vi "VIH HelpGen - Build HTML Help.vi"(6 "Allowed files (empty=all)":path[](array[path]), 8 "error in":errorcluster, 9 "File paths":path[](array[path]), 10 "Menu paths":path[](array[path]), 11 "Project Tree":T1) -> (0 "error out":errorcluster, 3 "dup Project Tree":T1)   [LabVIEW 2014]
doc: "::: VI Helpeks :::\nCopyright (c) 2000-2026 Konstantin Shifershteyn. All rights reserved."
uses:
  _VIH Project Manager.llb/VIH Project Tree Typedef - Tree Refnum.ctl
  _VIH HelpGen - Palette.llb/VIH HelpGen Typedef - Palette - Item Info Cluster.ctl
  _VIH HelpGen - Palette.llb/VIH HelpGen Typedef - Palette - Item Type Enum.ctl
panel:
  # "VI Helpeks\nCopyright (c) 2012-2026 Konstantin Shifershteyn"
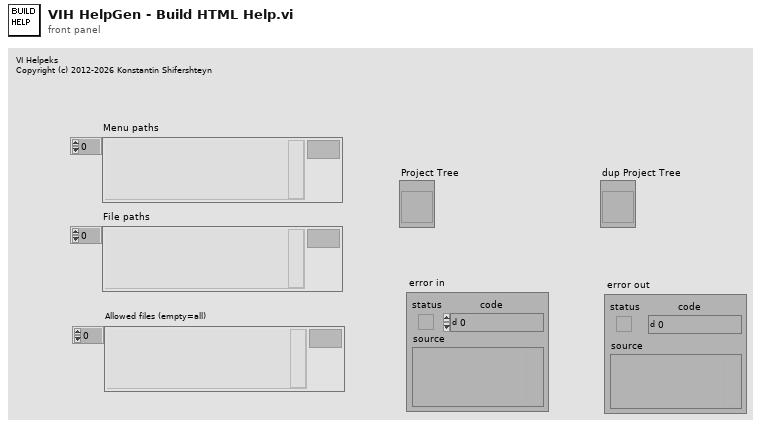
[diagram p1: front panel]
types:
  T1 = typedef "VIH Project Tree Typedef - Tree Refnum.ctl" = refnum<vi>
  T2 = enum16{"nop", "Start", "Stop", "Run-prep", "Run-VI", "Run-Menu"}
  T3 = typedef "VIH HelpGen Typedef - Palette - Item Info Cluster.ctl" = cluster{"Item Type":T4, "Item Name":string, "Item File":path, "Parent palette":path, "Not found":bool}
  T4 = typedef "VIH HelpGen Typedef - Palette - Item Type Enum.ctl" = enum32{"<Invalid>", "<unknown>", "VI", "Menu", "LV Func", "Express VI", "Poly VI", "CTL", "HTML"}
  T5 = cluster{"Show Window":bool, "Show Progress":bool, "Generate HTML":bool, "Generate HHP":bool, "Generate CHM":bool}
  T6 = typedef "VIH - CHM Project - HHP Generation Params Cluster.ctl" = cluster{"HHP_Template":enum16{"default", "custom"}, "HHP_Template_CustomPath":path, "HHP_Target":enum16{"default", "custom"}, "HHP_Target_CustomPath":path, "HHP_CreateTOC":bool, "HHP_CreateIDX":bool, "HHP_DefaultTopic":enum16{"auto", "custom"}, "HHP_DefaultTopic_CustomPath":path, "CHM_Filename":path, "HHP_AutoBuild":bool, "CHM_AutoBuild":bool}
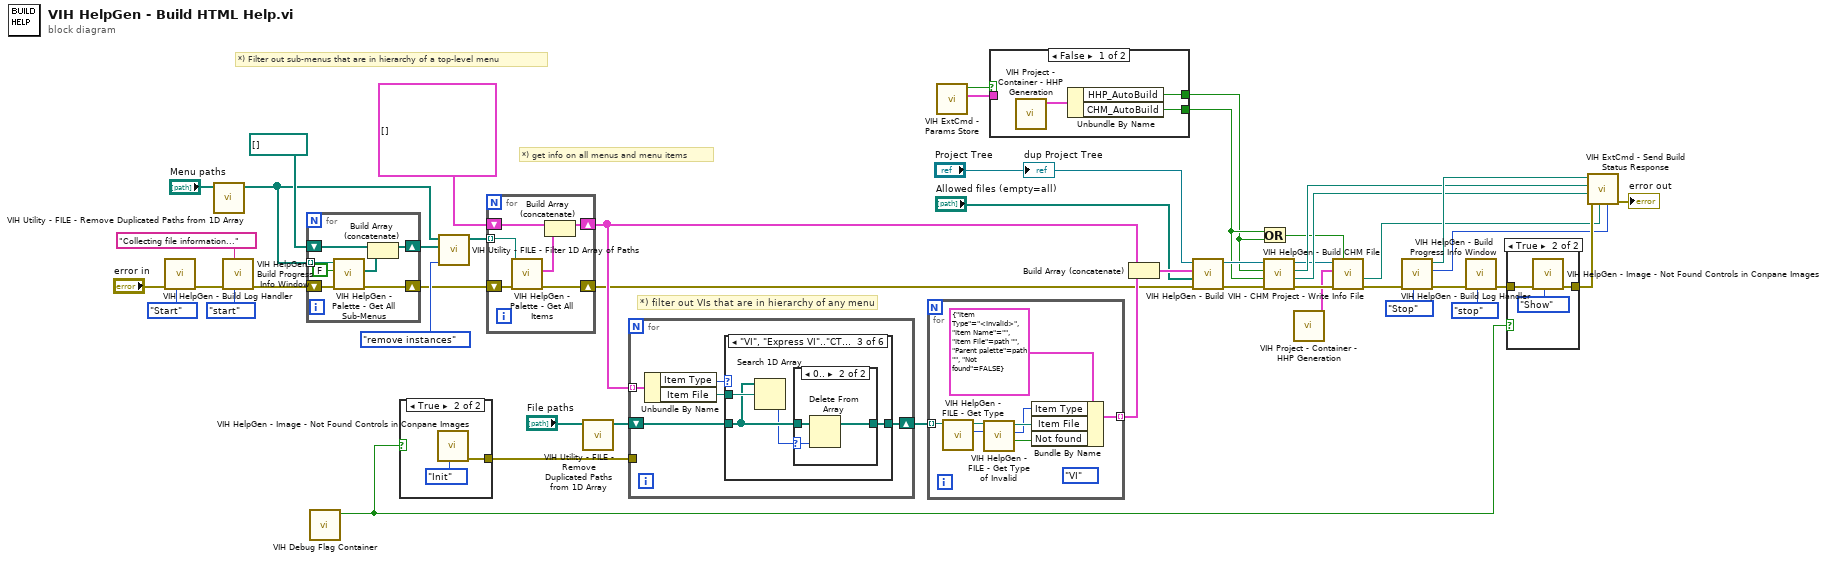
[diagram p0: block diagram]
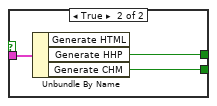
[diagram p2: hidden frame]
diagram:
  # "*) filter out VIs that are in hierarchy of any menu"
  # "*) get info on all menus and menu items"
  # "*) Filter out sub-menus that are in hierarchy of a top-level menu"
  n1 = call "VIH HelpGen - Build Log Handler.vi"("cmd (nop)"=T2."Start" ("cmd"), "error in"="error in") -> ("error out"=w35:errorcluster)  [unwired: 5 in, 4 out]
  n2 = call "VIH Utility - FILE - Remove Duplicated Paths from 1D Array.vi"("Array in"="Menu paths") -> ("Array out"=w28:path[])  [unwired: 9 in, 1 out]
  n3 = call "VIH HelpGen - Build Progress Info Window.vi"("Mode (run1)"=enum16{"start", "stop", "run1", "run2"}."start" ("Mode (run)"), "Message"="Collecting file information...", "error in"=w35) -> ("error out"=w33:errorcluster)  [unwired: 8 in]
  n4 = for {
    tunnel: w28 -> [w54] mode=indexing
    shift-right: [w51] -> w32
    shift-left: path[] [] -> [w52]
    shift-right: [w49] -> w27
    shift-left: w33 -> [w50]
    n5 = call "VIH HelpGen - Palette - Get All Sub-Menus.vi"("error in"=w50, "Include master menu (T)"=FALSE, "Palette Path"=w54) -> ("error out"=w49:errorcluster, "Palette Paths"=w53:path[])  [unwired: 7 in]
    n6 = Build Array (concatenate)(w52, w53) -> (w51:path[])
  }
  n7 = call "VIH Debug Flag Container.vi"() -> ("Debug Mode"=w23:bool)  [unwired: 11 in]
  n8 = case shown="True" w23 {
    tunnel: [_ w55] -> w26
    frame False {
    }
    frame True {
      n9 = call "VIH HelpGen - Image - Not Found Controls in Conpane Images.vi"("cmd"=enum16{"nop", "Init", "Add", "Show"}."Init") -> ("error out"=w55:errorcluster)  [unwired: 10 in]
    }
  }
  n10 = call "VIH Utility - FILE - Filter 1D Array of Paths.vi"("Action (keep instances)"=enum16{"keep instances", "remove instances"}."remove instances", "Instances"=w32, "Paths in"=w28) -> ("Paths out"=w29:path[])  [unwired: 4 in]
  n11 = for {
    shift-right: [w60] -> w39
    shift-left: w27 -> [w62]
    tunnel: w29 -> [w61] mode=indexing
    shift-right: [w57] -> w45
    shift-left: T3[] [] -> [w58]
    n12 = call "VIH HelpGen - Palette - Get All Items.vi"("error in"=w62, "Palette Path"=w61) -> ("error out"=w60:errorcluster, "Items Array"=w59:T3[])  [unwired: 7 in, 1 out]
    n13 = Build Array (concatenate)(w58, w59) -> (w57:T3[])
  }
  n14 = call "VIH Utility - FILE - Remove Duplicated Paths from 1D Array.vi"("Array in"="File paths") -> ("Array out"=w40:path[])  [unwired: 9 in, 1 out]
  n15 = for {
    tunnel: w45 -> [w67] mode=indexing
    shift-right: [w63] -> w46
    shift-left: w40 -> [w64]
    tunnel: w26 -> [_]
    n16 = Unbundle By Name(w67) -> ("Item Type"=w66:T4, "Item File"=w65:path)
    n17 = case shown="\"VI\", \"Express VI\"..\"CTL\"" w66 {
      tunnel: w65 -> [_ _ w73 _ _ _]
      tunnel: w64 -> [w68 w69 w72 w78 w79 w80]
      tunnel: [w68 w69 w71 w78 w79 w80] -> w63
      frame "<Invalid>" {
      }
      frame "<unknown>" {
      }
      frame "VI", "Express VI".."CTL" {
        n18 = Search 1D Array(1D array=w72, element=w73) -> (index of element=w70:i32)  [unwired: 1 in]
        n19 = case shown="0.." w70 {
          selector: w70 -> [_ w75]
          tunnel: w72 -> [w74 w77]
          tunnel: [w74 w76] -> w71
          frame ..-1 {
          }
          frame 0.. {
            n20 = Delete From Array "Delete From Array"(array=w77, index=w75) -> (array with subset deleted=w76:path[])  [unwired: 1 in, 1 out]
          }
        }
      }
      frame "Menu" {
      }
      frame "LV Func" {
      }
      frame "HTML" {
      }
    }
  }
  n21 = for {
    tunnel: w46 -> [w87] mode=indexing
    tunnel: [w88] -> w44 mode=indexing
    (unwired) VIH_HelpGen_Typedef_-_Palette_-_Item_Type_Enum."VI" ("Item Type")
    n22 = call "VIH HelpGen - FILE - Get Type.vi"("File Path"=w87) -> ("File Type"=w84:T4, "dup File Path"=w85:path)  [unwired: 8 in, 1 out]
    n23 = call "VIH HelpGen - FILE - Get Type of Invalid.vi"("File Type"=w84, "File Path"=w85) -> ("Not found"=w82:bool, "File Type out"=w81:T4, "File Path out"=w83:path)  [unwired: 6 in, 1 out]
    n24 = Bundle By Name(cluster=T3 {"Item Type"=enum."<Invalid>", "Item Name"="", "Item File"=path "", "Parent palette"=path "", "Not found"=FALSE} ("Item Info"), "Item Type"=w81, "Item File"=w83, "Not found"=w82) -> (w88:T3)
  }
  n25 = call "VIH ExtCmd - Params Store.vi"() -> ("Params"=w15:T5, "Ext Command"=w12:bool)  [unwired: 10 in]
  n26 = case shown="False" w12 {
    tunnel: w15 -> [_ w94]
    tunnel: [w90 w93] -> w3
    tunnel: [w89 w92] -> w4
    frame False {
      n27 = call "VIH Project - Container - HHP Generation.vi"() -> ("HHP_Generation out"=w91:T6)  [unwired: 11 in]
      n28 = Unbundle By Name(w91) -> ("HHP_AutoBuild"=w90:bool, "CHM_AutoBuild"=w89:bool)
    }
    frame True {
      n29 = Unbundle By Name(w94) -> ("Generate HHP"=w93:bool, "Generate CHM"=w92:bool)  [unwired: 1 out]
    }
  }
  n30 = Build Array (concatenate)(w45, w44) -> (w25:T3[])
  n31 = call "VIH HelpGen - Build.vi"("error in"=w39, "Allowed files"="Allowed files (empty=all)", "Items Array"=w25, "Project Tree"="Project Tree") -> ("error out"=w14:errorcluster, "dup Project Tree"=w6:T1)  [unwired: 5 in, 1 out]
  n32 = Or(x=w4, y=w3) -> (x .or. y?=w2:bool)
  n33 = call "VIH HelpGen - Build CHM File.vi"("error in"=w14, "Compile CHM file"=w4, "Create HHP file"=w3, "Project Tree"=w6) -> ("error out"=w10:errorcluster, "CHM File path"=w16:path, "HHP File path"=w17:path, "dup Project Tree"=w9:T1)  [unwired: 4 in]
  n34 = call "VIH Project - Container - HHP Generation.vi"() -> ("HHP_Generation out"=w5:T6)  [unwired: 11 in]
  n35 = call "VIH - CHM Project - Write Info File.vi"("Expect HHP exist (T)"=w2, "error in"=w10, "HHP_Generation"=w5, "Project Tree"=w9) -> ("error out"=w8:errorcluster, "Info File"=w1:path)  [unwired: 4 in, 2 out]
  n36 = call "VIH HelpGen - Build Log Handler.vi"("cmd (nop)"=T2."Stop" ("cmd"), "error in"=w8) -> ("error out"=w13:errorcluster, "errors"=w11:i32, "log file path"=w18:path)  [unwired: 5 in, 2 out]
  n37 = call "VIH HelpGen - Build Progress Info Window.vi"("Mode (run1)"=enum16{"start", "stop", "run1", "run2"}."stop" ("Mode (run)"), "error in"=w13) -> ("error out"=w21:errorcluster)  [unwired: 9 in]
  n38 = case shown="True" w23 {
    tunnel: w21 -> [w95 w97]
    tunnel: [w95 w96] -> w19
    frame False {
    }
    frame True {
      n39 = call "VIH HelpGen - Image - Not Found Controls in Conpane Images.vi"("cmd"=enum16{"nop", "Init", "Add", "Show"}."Show", "error in"=w97) -> ("error out"=w96:errorcluster)  [unwired: 9 in]
    }
  }
  n40 = call "VIH ExtCmd - Send Build Status Response.vi"("Errors"=w11, "Help Info file"=w1, "error in"=w19, "CHM file"=w16, "HHP file"=w17, "HTML Build Log file"=w18) -> ("error out"=→"error out":errorcluster)  [unwired: 5 in]
  "dup Project Tree" <- "Project Tree"
